vi "VIH Utility - APP - Generic Error Handler.vi"(6 "nesting level":i32, 8 "error in":errorcluster, 9 "error reason":string, 10 "error location":string, 11 "error code":i32) -> (0 "error out":errorcluster, 3 "error":bool)   [LabVIEW 2014]
doc: "::: VI Helpeks :::\nCopyright (c) 2000-2026 Konstantin Shifershteyn. All rights reserved."
panel:
  # "VI Helpeks\nCopyright (c) 2012-2026 Konstantin Shifershteyn"
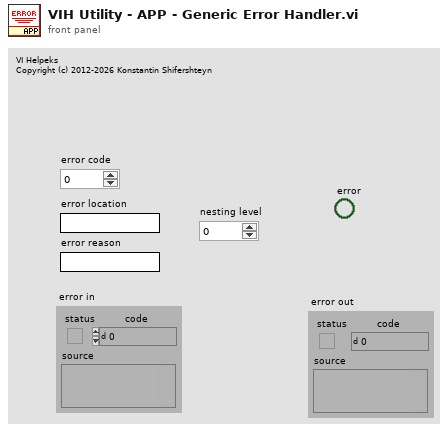
[diagram p1: front panel]
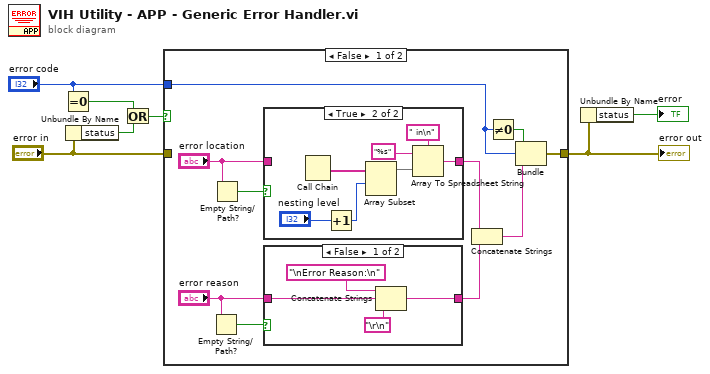
[diagram p0: block diagram]
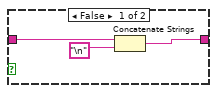
[diagram p3: hidden frame]
diagram:
  n1 = Equal To 0?(x="error code") -> (x = 0?=w6:bool)
  n2 = Unbundle By Name("error in") -> ("status"=w7:bool)
  n3 = Or(x=w6, y=w7) -> (x .or. y?=w3:bool)
  n4 = case shown="False" w3 {
    tunnel: "error code" -> [w14 _]
    tunnel: "error in" -> [_ w33]
    tunnel: [w15 w33] -> w1
    frame False {
      n5 = Empty String/Path?(string/path="error reason") -> (empty?=w12:bool)
      n6 = Empty String/Path?(string/path="error location") -> (empty?=w17:bool)
      n7 = case shown="True" w17 {
        tunnel: "error location" -> [w25 _]
        tunnel: [w24 w26] -> w10
        frame False {
          n8 = Concatenate Strings(w25, "\n" ("delimiter (Tab)")) -> (w24:string)
        }
        frame True {
          n9 = Call Chain() -> (call chain=w30:string[])
          n10 = Increment(x="nesting level") -> (x+1=w32:i32)
          n11 = Array Subset(array=w30, index=w32) -> (w29:string[])  [unwired: 1 in]
          n12 = Array To Spreadsheet String(delimiter (Tab)=" in\n", array=w29, 3:"%s" ("format string")) -> (spreadsheet string=w26:string)
        }
      }
      n13 = case shown="False" w12 {
        tunnel: "error reason" -> [w19 w22]
        tunnel: [w18 w22] -> w9
        frame False {
          n14 = Concatenate Strings("\nError Reason:\n", w19, "\r\n") -> (w18:string)
        }
        frame True {
        }
      }
      n15 = Concatenate Strings(w10, w9) -> (w8:string)
      n16 = Not Equal To 0?(x=w14) -> (x != 0?=w13:bool)
      n17 = Bundle(w13, "error code"=w14, w8) -> (w15:cluster{bool, "error code":i32, string})  [unwired: 1 out]
    }
    frame True {
    }
  }
  "error out" <- w1
  n18 = Unbundle By Name(w1) -> ("status"=→"error":bool)
